vi "LUV ou NEP.vi"(3 "Booléen":bool) -> (1 "Nom cuve":string)   [LabVIEW 2022 SP3]
uses:
  Variables globales/Variable glob generale.vi
  <vilib>/Utility/config.llb/NI_LVConfig.lvlib
panel:
  in  "Bouton OK":bool
  in  "Choisir":u16(ring) caption="Choisir le dossier principal :" items=["Ligne UV", "NEPTUNE"]
  # "spécificité LUV-NEP\nChoix du dossier principal"
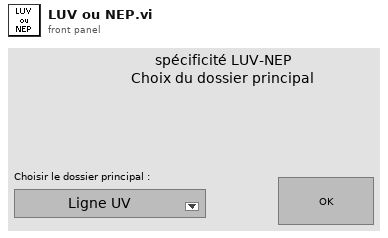
[diagram p1: front panel]
types:
  T1 = typedef "NI_LVConfig.lvlib/Config Data RefNum.ctl" = refnum<k1>
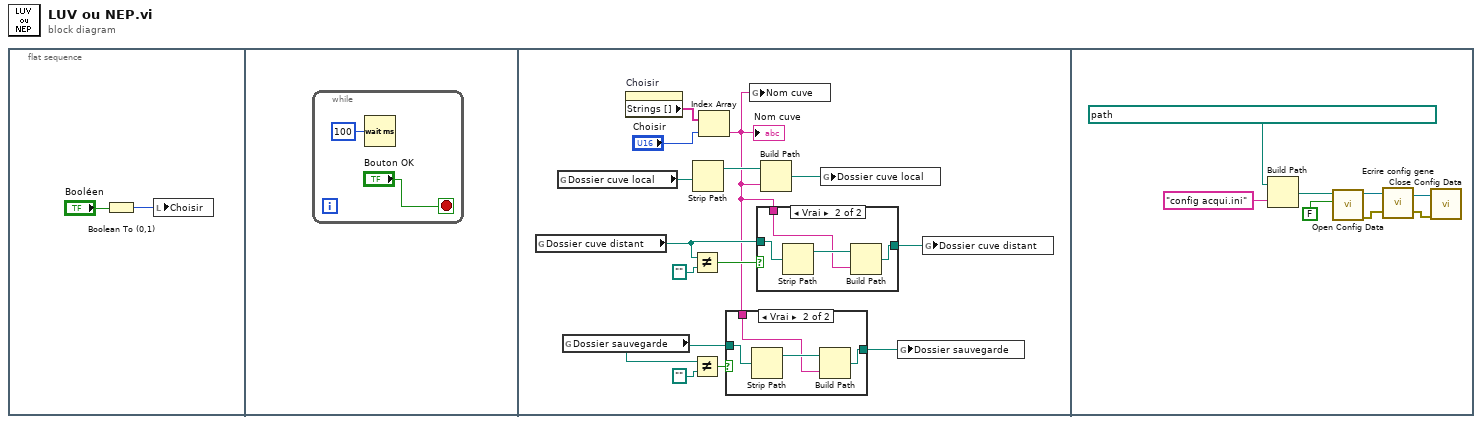
[diagram p0: block diagram]
diagram:
  n1 = flat-sequence {
    frame #0 {
      n2 = Boolean To (0,1)(Boolean="Booléen") -> (0, 1=w1:i16)
      n3 = local write "Choisir"(w1) -> ()
    }
    frame #1 {
      n4 = while {
        stop <- "Bouton OK" stop-if-true
        n5 = Wait (ms)(milliseconds to wait=u32 100 ("attente (ms)")) -> ()  [unwired: 1 out]
      }
    }
    frame #2 {
      n6 = global read "Variable glob generale.vi" "Dossier cuve distant"() -> (w11:path)
      n7 = global read "Variable glob generale.vi" "Dossier cuve local"() -> (w16:path)
      n8 = global read "Variable glob generale.vi" "Dossier sauvegarde"() -> (w7:path)
      n9 = property on="Choisir" class="MDér (strict)"() -> ("Strings []"=w18:string[])  [unwired: 2 in, 2 out]
      n10 = Not Equal?(x=w11, y=path "") -> (x != y?=w12:bool)
      n11 = Not Equal?(x=w7, y=path "") -> (x != y?=w8:bool)
      n12 = Strip Path(path=w16) -> (stripped path=w15:path)  [unwired: 1 out]
      n13 = Index Array(array=w18, index="Choisir") -> (element=w6:string)
      "Nom cuve" <- w6
      n14 = case shown="Vrai" w8 {
        tunnel: w7 -> [w19 w22]
        tunnel: w6 -> [_ w21]
        tunnel: [w19 w20] -> w5
        frame False {
        }
        frame True {
          n15 = Strip Path(path=w22) -> (stripped path=w23:path)  [unwired: 1 out]
          n16 = Build Path(base path=w23, name or relative path=w21) -> (appended path=w20:path)
        }
      }
      n17 = global write "Variable glob generale.vi" "Nom cuve"(w6) -> ()
      n18 = case shown="Vrai" w12 {
        tunnel: w11 -> [w24 w27]
        tunnel: w6 -> [_ w26]
        tunnel: [w24 w25] -> w10
        frame False {
        }
        frame True {
          n19 = Strip Path(path=w27) -> (stripped path=w28:path)  [unwired: 1 out]
          n20 = Build Path(base path=w28, name or relative path=w26) -> (appended path=w25:path)
        }
      }
      n21 = Build Path(base path=w15, name or relative path=w6) -> (appended path=w14:path)
      n22 = global write "Variable glob generale.vi" "Dossier cuve local"(w14) -> ()
      n23 = global write "Variable glob generale.vi" "Dossier sauvegarde"(w5) -> ()
      n24 = global write "Variable glob generale.vi" "Dossier cuve distant"(w10) -> ()
    }
    frame #3 {
      n25 = Build Path(base path=path "C:/LABVIEW/PRES+TEMP+REG dernière version/Configurations", name or relative path="config acqui.ini" ("nom ou chemin relatif")) -> (appended path=w34:path)
      n26 = call <vilib>:"Open Config Data.vi"("create file if necessary (T)"=FALSE ("create file if necessary? (T)"), "configuration file path"=w34) -> ("error out"=w32:errorcluster, "refnum"=w33:T1)  [unwired: 7 in, 1 out]
      n27 = call "Ecrire config gene.vi"("error in (no error)"=w32, "refnum"=w33) -> ("error out"=w30:errorcluster, "refnum out"=w31:T1)
      n28 = call <vilib>:"Close Config Data.vi"("error in (no error)"=w30, "refnum"=w31) -> ()  [unwired: 8 in, 2 out]
    }
  }
